vi "Chiller.vi"(6 "error in (no error)":errorcluster, 7 "dt (s)":dbl=1.0, 8 "Setpoint (C)":dbl, 9 "Action":T1) -> (0 "error out":errorcluster, 1 "Setpoit out (C)":dbl, 2 "Temp (C)":dbl)   [LabVIEW 2026]
uses:
  Typedefs/Chiller Action.ctl
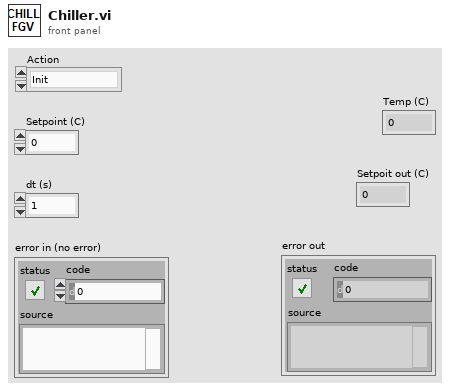
[diagram p1: front panel]
types:
  T1 = typedef "Chiller Action.ctl" = enum16{"Init", "Set Setpoint", "Step", "Read"}
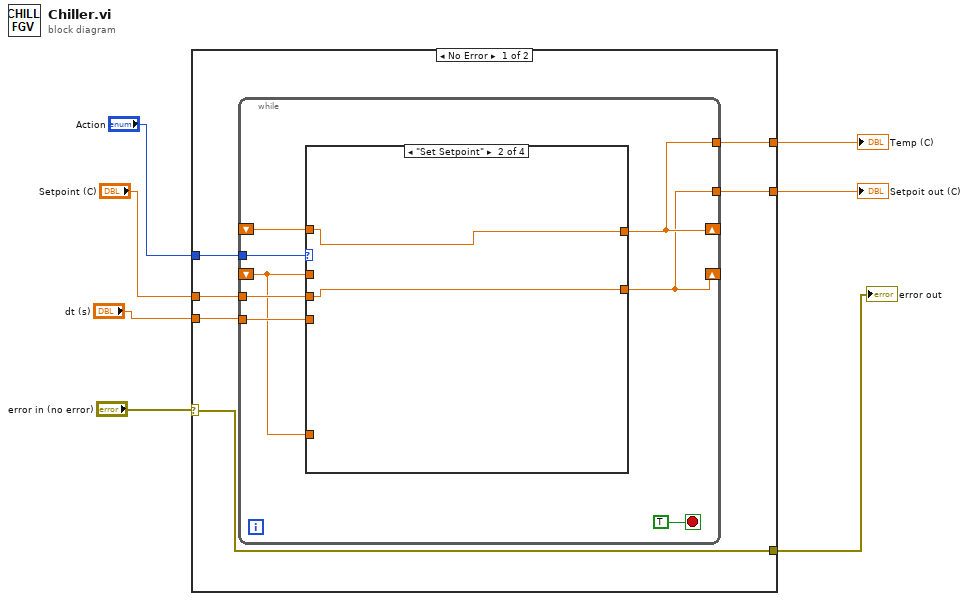
[diagram p0: block diagram]
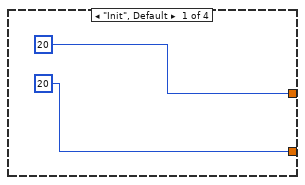
[diagram p2: hidden frame]
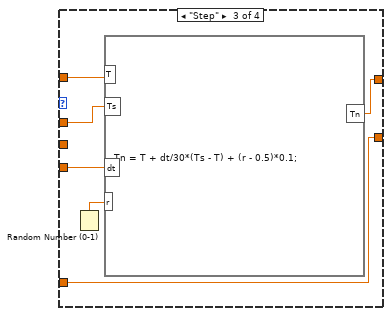
[diagram p3: hidden frame]
diagram:
  n1 = case shown="No Error" "error in (no error)" {
    selector: "error in (no error)" -> [w8 w34]
    tunnel: "Action" -> [w13 _]
    tunnel: "dt (s)" -> [w12 _]
    tunnel: [w11 _] -> w5
    tunnel: [w10 _] -> w4
    tunnel: "Setpoint (C)" -> [w9 _]
    tunnel: [w8 w34] -> w1
    frame No Error {
      n2 = while {
        shift-right: [w17] -> _
        shift-left: _ -> [w19]
        shift-right: [w16] -> _
        shift-left: _ -> [w14]
        tunnel: w13 -> [w20]
        tunnel: w12 -> [w18]
        tunnel: [w17] -> w11
        tunnel: [w16] -> w10
        tunnel: w9 -> [w15]
        stop <- TRUE stop-if-true
        n3 = case shown="\"Set Setpoint\"" w20 {
          tunnel: w19 -> [_ w25 w31 w33]
          tunnel: [20 w25 w29 w33] -> w17
          tunnel: [20 w24 w26 w32] -> w16
          tunnel: w18 -> [_ _ w30 _]
          tunnel: w14 -> [_ _ w27 w32]
          tunnel: w15 -> [_ w24 _ _]
          tunnel: w14 -> [_ _ w26 _]
          frame "Init", Default {
          }
          frame "Set Setpoint" {
          }
          frame "Step" {
            n4 = Random Number (0-1)() -> (number: 0 to 1=w28:dbl)
            n5 = formula code="Tn = T + dt/30*(Ts - T) + (r - 0.5)*0.1;"("T"=w31, "Ts"=w27, "dt"=w30, "r"=w28) -> ("Tn"=w29:dbl)
          }
          frame "Read" {
          }
        }
      }
    }
    frame Error {
    }
  }
  "Temp (C)" <- w5
  "Setpoit out (C)" <- w4
  "error out" <- w1
